vi "P3_RunVIAsync.vi"(11 "Inputs":string[](array[string])) -> (2 "Output/Failure":string, 3 "CLI Process Return Code":i32)   [LabVIEW 2026]
doc: "Slice 1.1 probe: Open VI Reference, Run VI with Wait until done FALSE, read Execution State, close the reference."
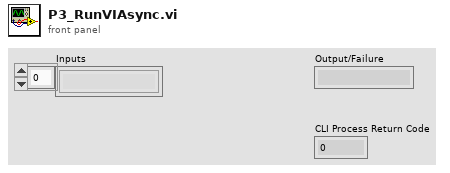
[diagram p1: front panel]
types:
  T1 = enum32{"Bad", "Idle", "Run top level", "Running"}
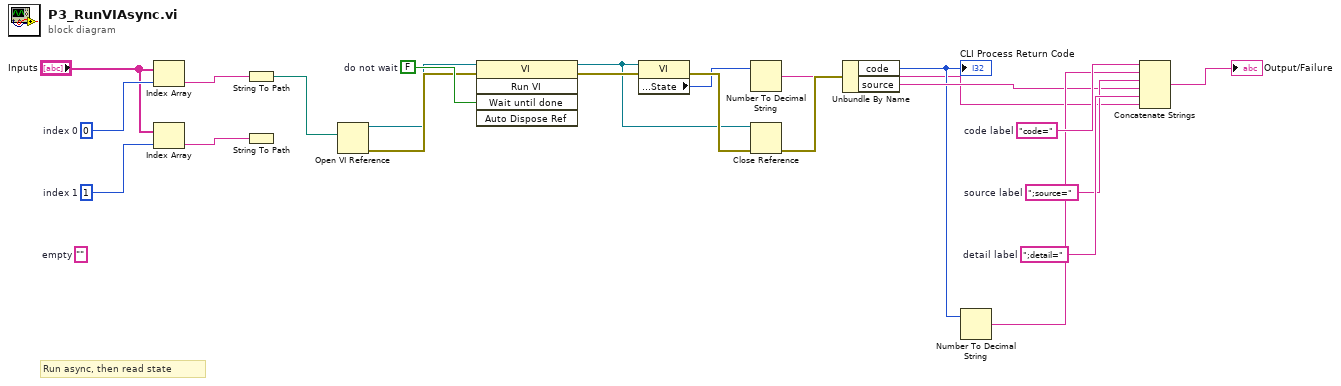
[diagram p0: block diagram]
diagram:
  w21 = ";detail="  # detail label
  w20 = ";source="  # source label
  w19 = "code="  # code label
  w9 = FALSE  # do not wait
  (unwired) ""  # empty
  w3 = 1  # index 1
  w2 = 0  # index 0
  # "Run async, then read state"
  n1 = Index Array(array="Inputs", index=w2) -> (element=w4:string)
  n2 = Index Array(array="Inputs", index=w3) -> (element=w5:string)
  n3 = String To Path(string=w4) -> (path=w6:path)
  n4 = String To Path(string=w5) -> ()  [unwired: 1 out]
  n5 = Open VI Reference(vi path=w6) -> (vi reference=w7:refnum<vi>, error out=w8:errorcluster)  [unwired: 5 in]
  n6 = invoke class="VI" method="Run VI"(reference=w7, error in=w8, "Wait until done"=w9) -> (reference out=w10:refnum<vi>, error out=w11:errorcluster)  [unwired: 2 in, 3 out]
  n7 = property class="VI"(reference=w10, error in=w11) -> (error out=w13:errorcluster, "Execution:State"=w12:T1)  [unwired: 1 out]
  n8 = Number To Decimal String(number=w12) -> (decimal integer string=w14:string)  [unwired: 1 in]
  n9 = Close Reference(reference=w10, error in (no error)=w13) -> (error out=w15:errorcluster)
  n10 = Unbundle By Name(w15) -> ("code"=w16:i32, "source"=w17:string)
  "CLI Process Return Code" <- w16
  n11 = Number To Decimal String(number=w16) -> (decimal integer string=w18:string)  [unwired: 1 in]
  n12 = Concatenate Strings(w19, w18, w20, w17, w21, w14) -> (→"Output/Failure":string)
